vi "csb warmup.vi"(7 "hdlc_state_size":i32, 8 "error in (no error)":errorcluster, 9 "hdlc_state":u8[](array[numeric]), 10 "ws_state_size":i32, 11 "ws_state":u8[](array[numeric])) -> (0 "error out":errorcluster, 1 "hdlc_state out":u8[](array[numeric]), 2 "function return":i32, 3 "ws_state out":u8[](array[numeric]))   [LabVIEW 2021, in "CANsub_Codec.lvlib"]
doc: "int32_t csb_warmup(uint8_t *ws_state, int32_t ws_state_size,\n uint8_t *hdlc_state, int32_t hdlc_state_size);"
uses:
  CANsub_Codec.lvlib
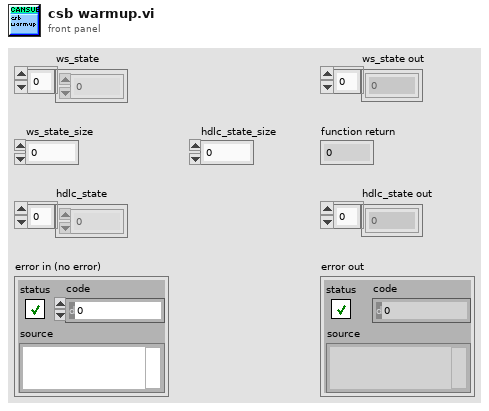
[diagram p1: front panel]
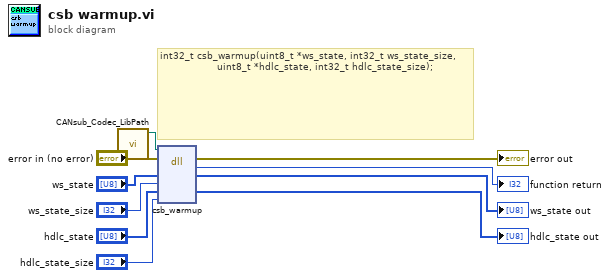
[diagram p0: block diagram]
diagram:
  # "int32_t csb_warmup(uint8_t *ws_state, int32_t ws_state_size,\n                   uint8_t *hdlc_state, int32_t hdlc_state_size);"
  n1 = call "CANsub_Codec_LibPath.vi"() -> ("Path"=w1:path)  [unwired: 11 in]
  n2 = dll-call lib="libcansub_codec.*" fn="csb_warmup"(path in=w1, error in="error in (no error)", "ws_state"="ws_state", "ws_state_size"="ws_state_size", "hdlc_state"="hdlc_state", "hdlc_state_size"="hdlc_state_size") -> (error out=→"error out":errorcluster, "return type"=→"function return":i32, "ws_state"=→"ws_state out":u8[], "hdlc_state"=→"hdlc_state out":u8[])  [unwired: 3 in, 1 out]
